vi "CSM - Mermaid - DebugTool.vi"() -> ()   [LabVIEW 2020]
doc: "Show CSM relationship Graph with mermaid"
uses:
  <vilib>/sklein/WebView2 XControl/WebView2 XControl/WebView2 Control.xctl
  <userlib>/_NEVSTOP/Communicable State Machine(CSM)/_Support/Typedef/_CSM_GlobalLog_MSG.ctl
  <userlib>/_NEVSTOP/Communicable State Machine(CSM)/_Support/Typedef/_CSM_Response Source Message.ctl
  <userlib>/_NEVSTOP/Communicable State Machine(CSM)/_Support/Typedef/_CSM_GlobalLog_MSG_TYPE.ctl
  <userlib>/_NEVSTOP/Communicable State Machine(CSM)/_tool/_debugConsole/_BroadcastDef.ctl
  <userlib>/_NEVSTOP/Communicable State Machine(CSM)/AdvanceAPI/CSM - Convert Error to Argument.vi
  <userlib>/_NEVSTOP/Communicable State Machine(CSM)/_Support/GlobalEvent/GEvt-Generate with Rule Check.vi
  <userlib>/_NEVSTOP/Communicable State Machine(CSM)/_Support/GlobalEvent/Cache-GEvt Refs.vi
  <userlib>/_NEVSTOP/Communicable State Machine(CSM)/AdvanceAPI/CSM - Make String Arguments Safe.vi
  <userlib>/_NEVSTOP/Communicable State Machine(CSM)/_Support/ChangeFlag/FlagInstance-GEvt Refs.vi
  <userlib>/_NEVSTOP/Communicable State Machine(CSM)/AdvanceAPI/CSM - Keywords.vi
  <userlib>/_NEVSTOP/Communicable State Machine(CSM)/_Support/ChangeFlag/ChangeFlag-Read.vi
  <userlib>/_NEVSTOP/Communicable State Machine(CSM)/_Polymophic/Add State(s) to Queue By BOOL(Element).vi
  <userlib>/_NEVSTOP/Communicable State Machine(CSM)/_Support/ChangeFlag/ChangeFlagDB.vi
  <userlib>/_NEVSTOP/Communicable State Machine(CSM)/_Support/GlobalEvent/FGV-GlobalEventRef(lvlibp).vi
  <userlib>/_NEVSTOP/Communicable State Machine(CSM)/_Support/GlobalEvent/FGV-GlobalEventQueues(lvlibp).vi
  <userlib>/_NEVSTOP/Communicable State Machine(CSM)/_Support/GlobalEvent/GEvt-Valid Subscribers.vi
  <userlib>/_NEVSTOP/Communicable State Machine(CSM)/_Support/GlobalEvent/LogFilter/LogFilter - Check.vi
  <userlib>/_NEVSTOP/Communicable State Machine(CSM)/_csmHelper/API/Create From VI Reference.vi
  <userlib>/_NEVSTOP/Communicable State Machine(CSM)/_csmHelper/API/Destroy.vi
  <userlib>/_NEVSTOP/Communicable State Machine(CSM)/_Support/GlobalEvent/LogFilter/LogFilter.lvclass
  <userlib>/_NEVSTOP/Communicable State Machine(CSM)/Communicable State Machine.lvlib
  _support/CSM Mermaid Support.lvlib
  <userlib>/_NEVSTOP/Communicable State Machine(CSM)/_csmHelper/CSM-Helper.lvclass
  <userlib>/_NEVSTOP/Communicable State Machine(CSM)/_tool/_file/csm-file-support.lvlib
  <userlib>/_NEVSTOP/Communicable State Machine(CSM)/_tool/_ui/csm-ui-support.lvlib
  <userlib>/_NEVSTOP/Communicable State Machine(CSM)/_tool/_csmlite/_csmlite.lvlib
  <userlib>/_NEVSTOP/Communicable State Machine(CSM)/_tool/_debugConsole/DebugConsole.lvlib
panel:
  in  "CSM":string(combo)
  in  "Search Button":bool
  in  "Draw Mermaid":bool
  in  "Type":T1(ring)
  in  "Tab":T2(tab)
  out "mermaid string":string
  in  "WebView2 Control":string(xcontrol)
  # "https://mermaid.live/"
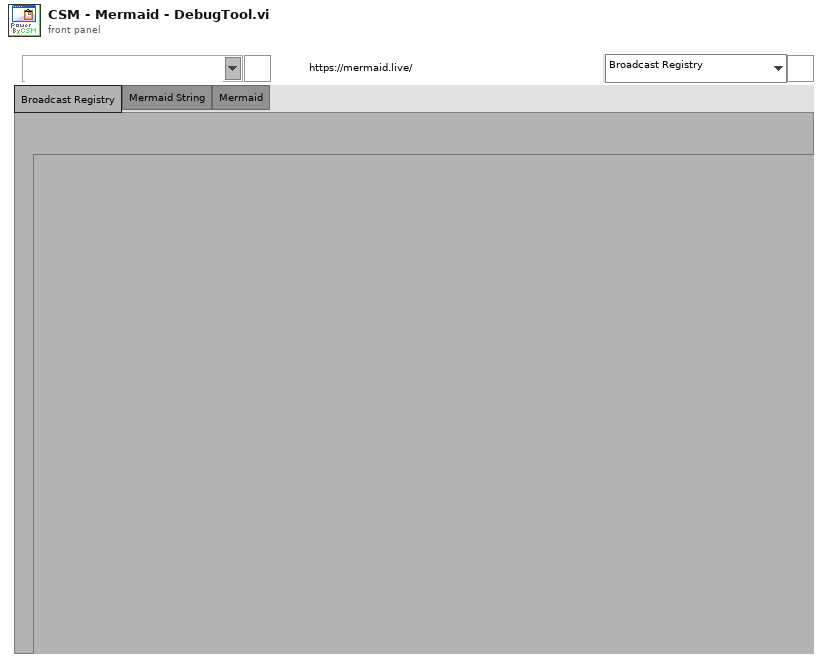
[diagram p1: front panel]
types:
  T1 = enum16{"Broadcast Registry", "CSM Interface", "CSM All Interfaces"}
  T2 = enum32{"Broadcast Registry", "Mermaid String", "Mermaid"}
  T3 = typedef "Communicable State Machine.lvlib/_CSM_GlobalLog_MSG.ctl" = cluster{"Name (\"\" to Use UUID)":string, "Current State":string, "Arguments":string, "Source Message":T4, "Source Module":string, "Complete(T)/Start(F)":bool, "LogType":T5, "Time Stamp":timestamp}
  T4 = typedef "Communicable State Machine.lvlib/_CSM_Response Source Message.ctl" = cluster{"‘State":string, "’Arguments":string, "’Error":errorcluster}
  T5 = typedef "Communicable State Machine.lvlib/_CSM_GlobalLog_MSG_TYPE.ctl" = enum16{"User Log", "State Change", "Status", "Interrupt", "Register", "Unregister", "Error Log", "Module Created", "Module Destroyed", "Async Message", "No-Rep Async Message", "Sync Message"}
  T6 = enum32{"Broadcast Registry", "Mermaid String", "Mermaid", "Error History"}
  T7 = enum32{"Invalid", "Standard", "Closed", "Hidden", "Minimized", "Maximized"}
  T8 = enum32{"invalid app kind", "Development System", "Run Time System", "Student Edition", "Embedded LabVIEW", "Evaluation", "Custom"}
  T9 = typedef "DebugConsole.lvlib/_BroadcastDef.ctl" = enum16{"<no action>", "Macro: Exit", "CSM: Module List Changed", "CSM: Scripts Changed", "CSM: Registration Changed", "CSM: Module Selected", "CSM: Message Excuted", "CSM: Broadcast Excuted", "CSM: Registration Action Excuted", "UI: Try to Change Command"}
  T10 = cluster{"Event Registration Refnum":refnum<event-registration>, "Event Registration Refnum":refnum<event-registration>}
  T11 = cluster{"Shift":bool, "Ctrl":bool, "Alt":bool, "Cmd":bool, "Opt":bool}
  T12 = cluster{"Core":cluster{"Current VI Reference":refnum<vi>, "Close Panel on Exit?":bool}, "Toolbar.Advance":refnum<vi>[], "LoggerWatchDogQueue":refnum<queue>, "LogFile":path, "Mermaid":cluster{"Template":string, "output path":path, "string":string}}
  T13 = cluster{"Template":string, "output path":path, "string":string}
  T14 = cluster{"Current VI Reference":refnum<vi>, "Close Panel on Exit?":bool}
  T15 = cluster{"Left":i32, "Right":i32, "Height":i32, "Width":i32}
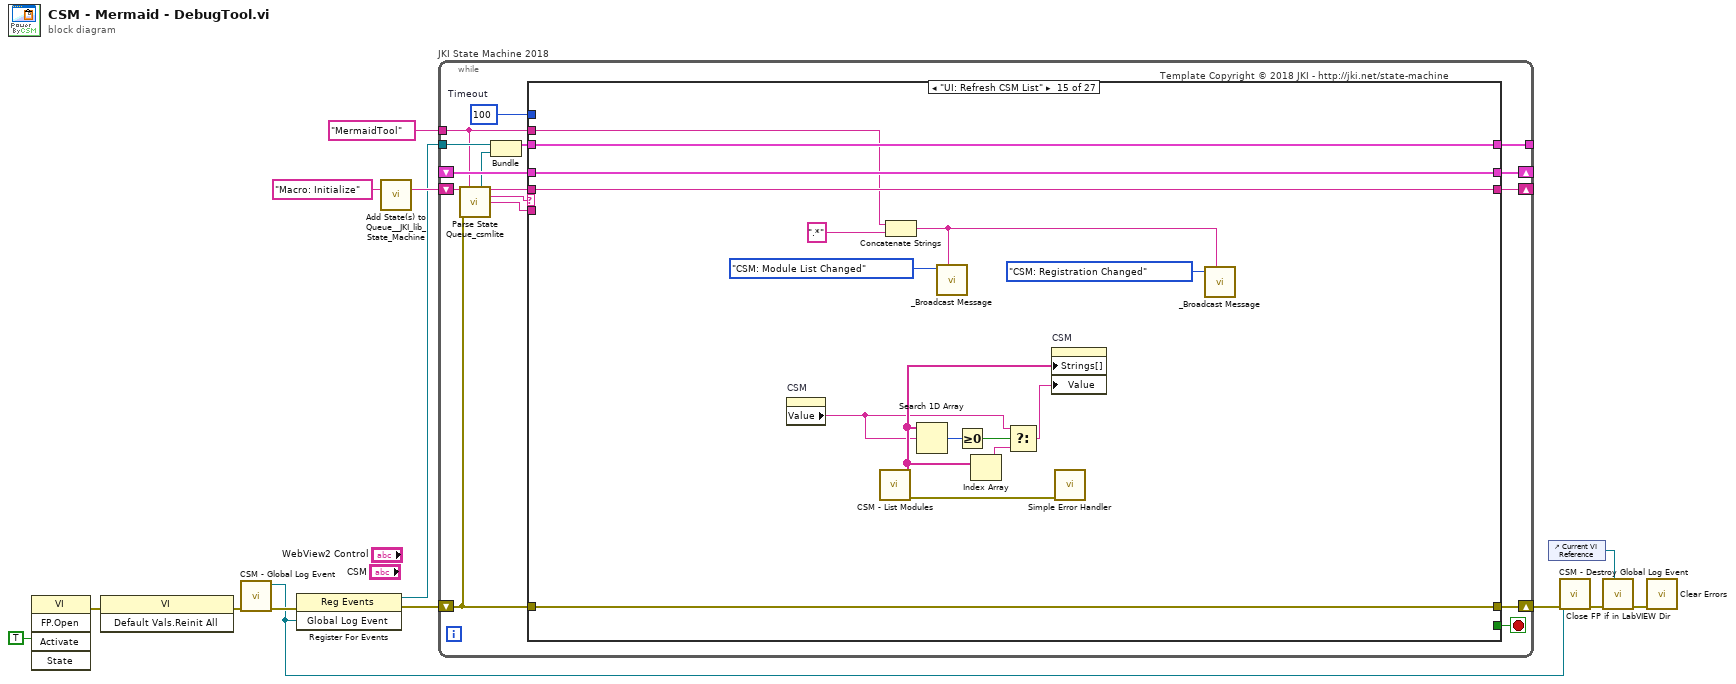
[diagram p0: block diagram]
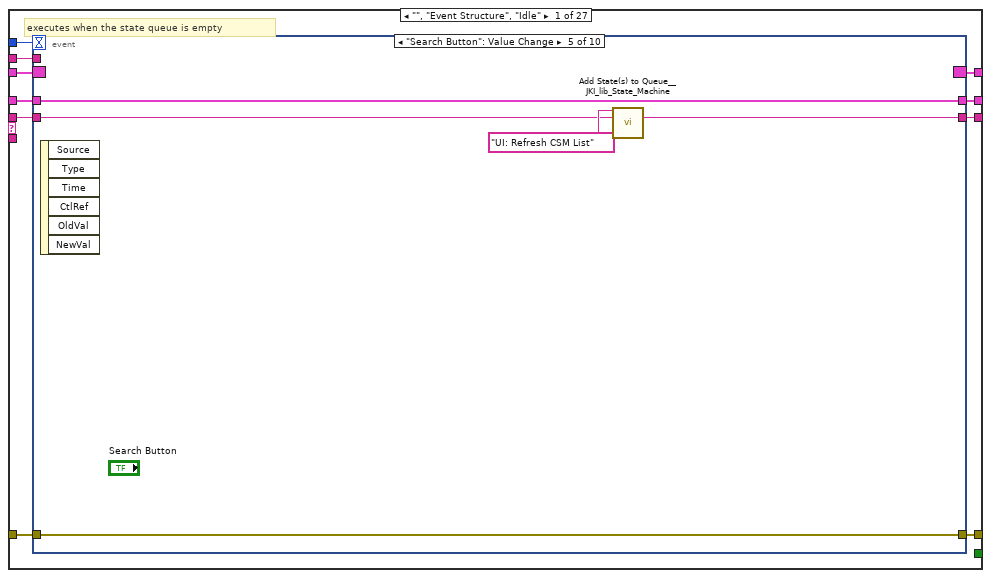
[diagram p2: hidden frame]
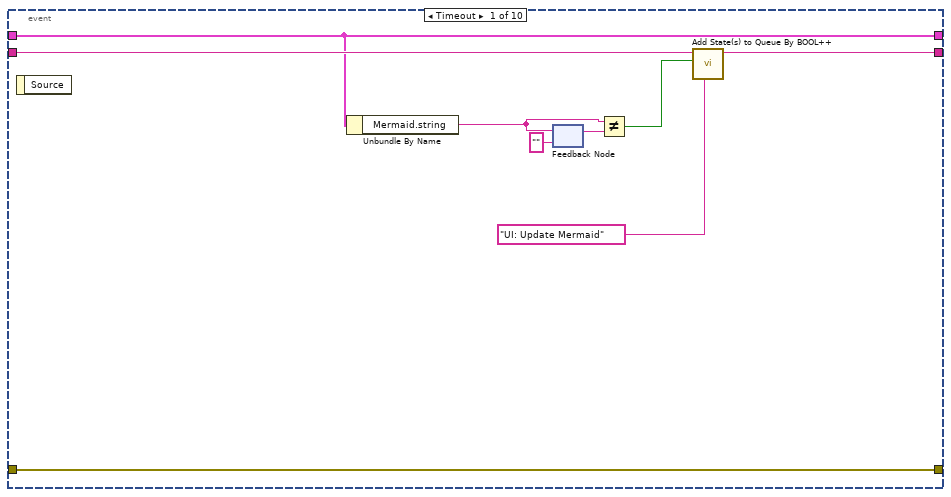
[diagram p3: hidden frame]
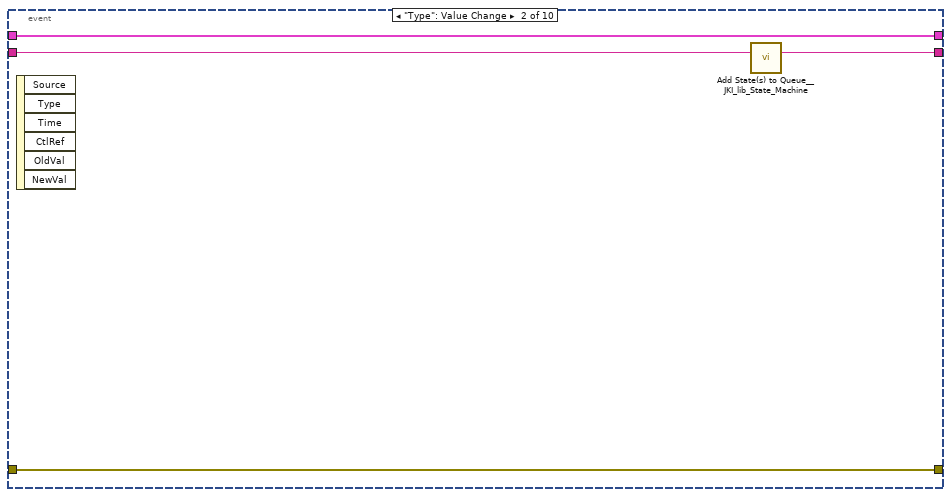
[diagram p4: hidden frame]
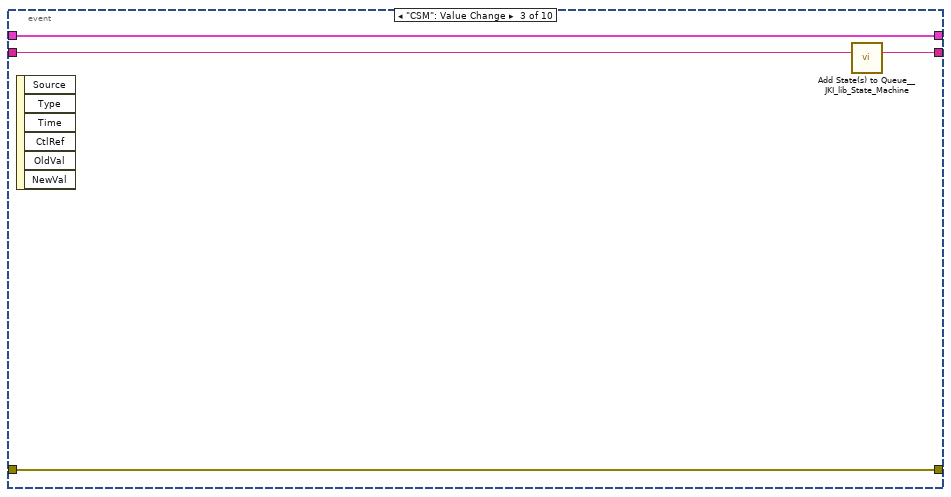
[diagram p5: hidden frame]
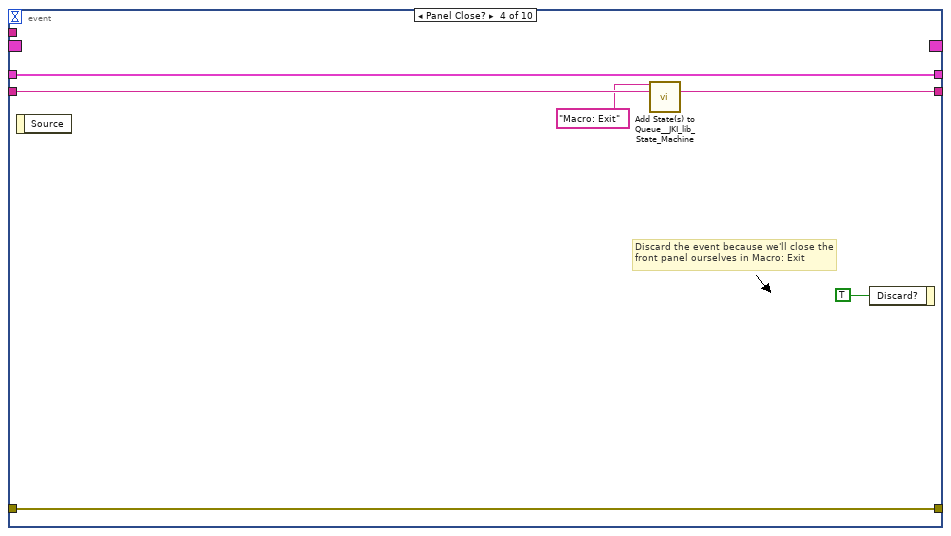
[diagram p6: hidden frame]
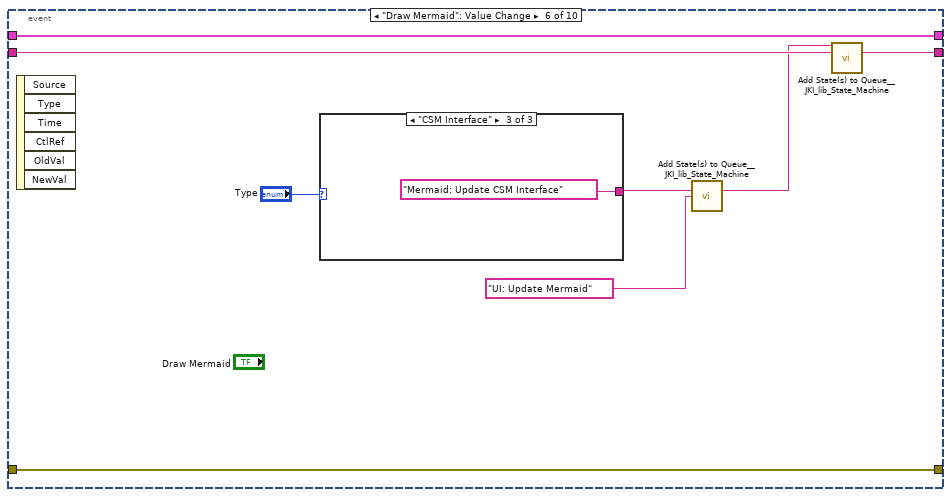
[diagram p7: hidden frame]
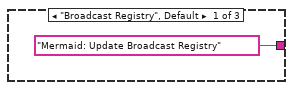
[diagram p8: hidden frame]
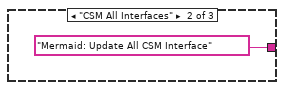
[diagram p9: hidden frame]
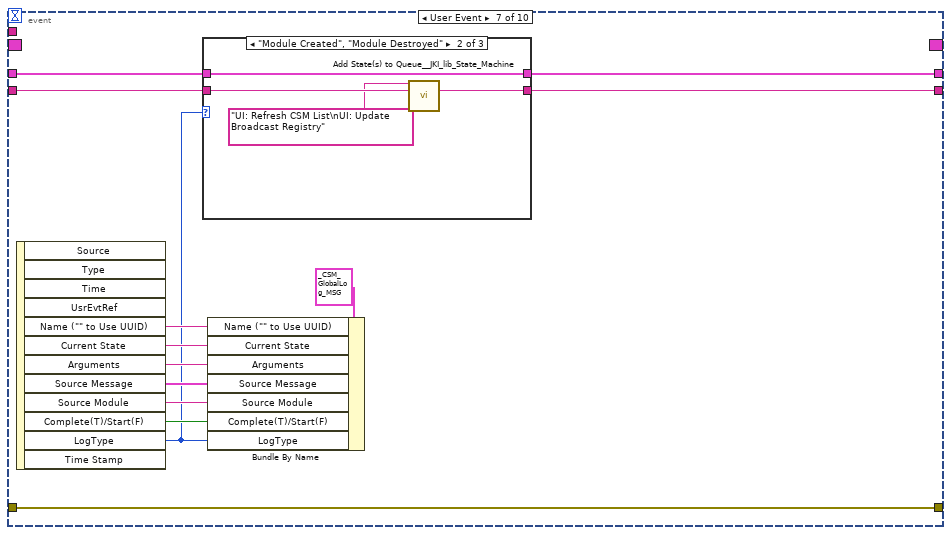
[diagram p10: hidden frame]
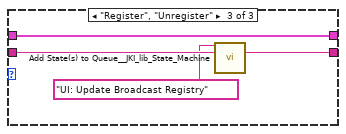
[diagram p12: hidden frame]
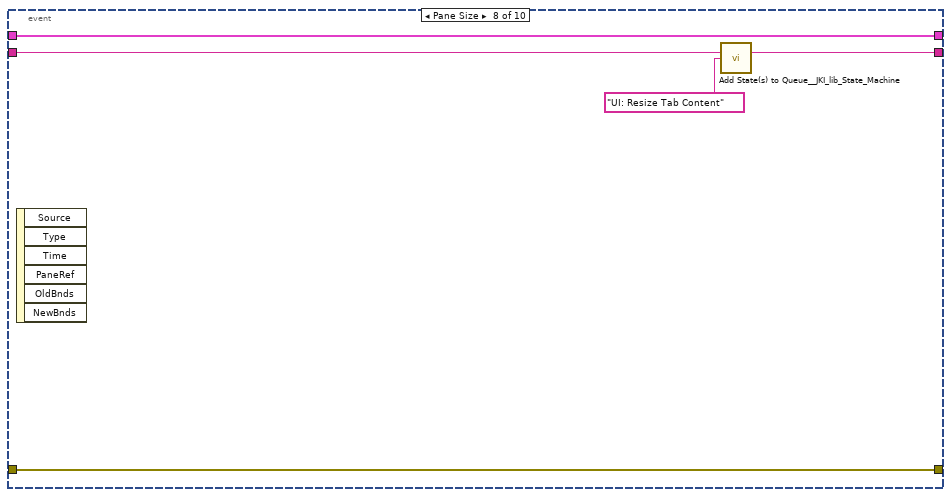
[diagram p13: hidden frame]
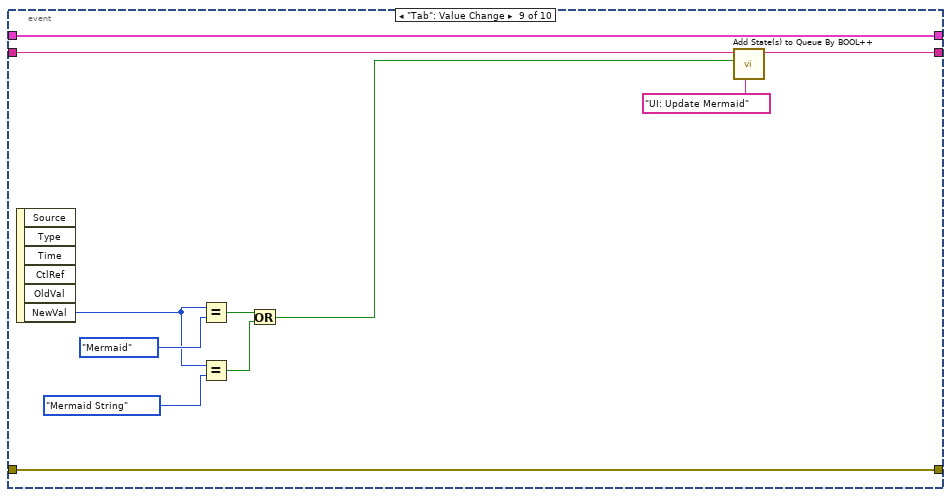
[diagram p14: hidden frame]
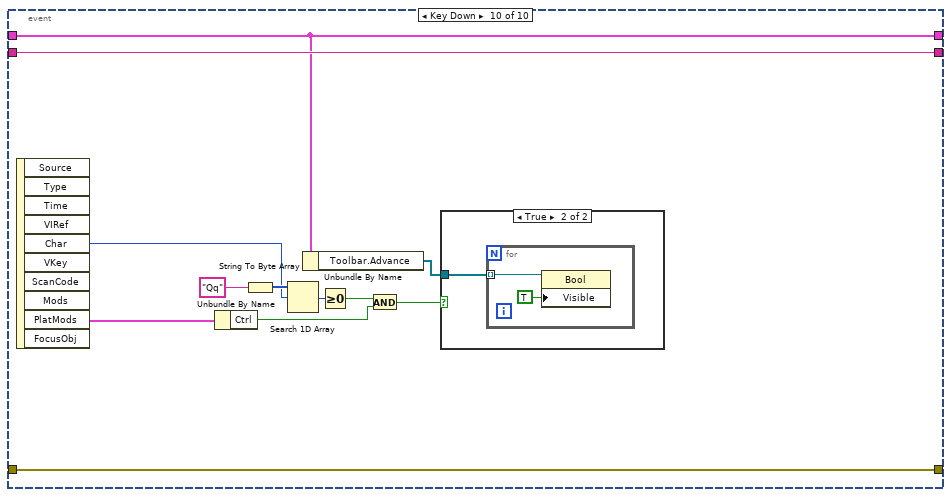
[diagram p15: hidden frame]
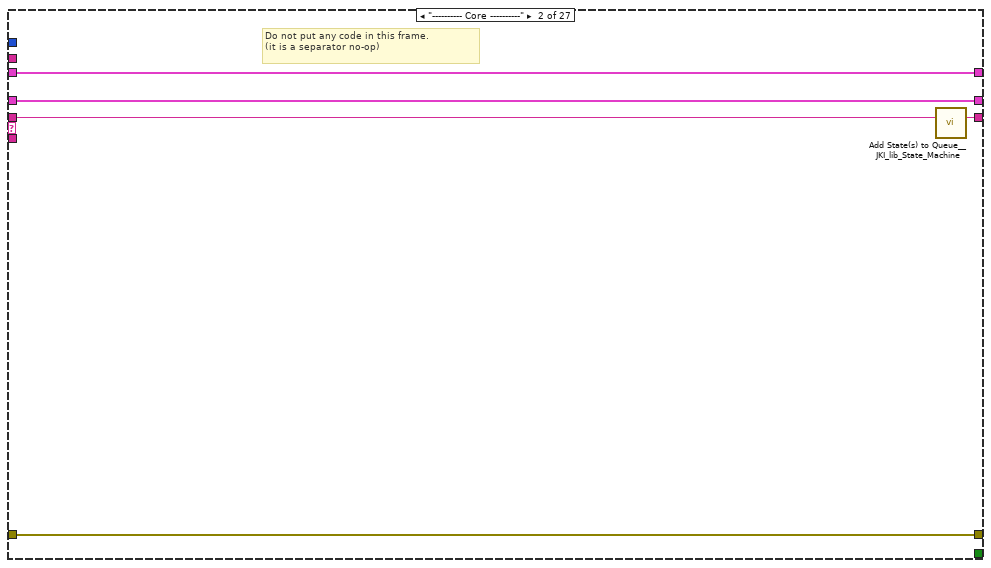
[diagram p17: hidden frame]
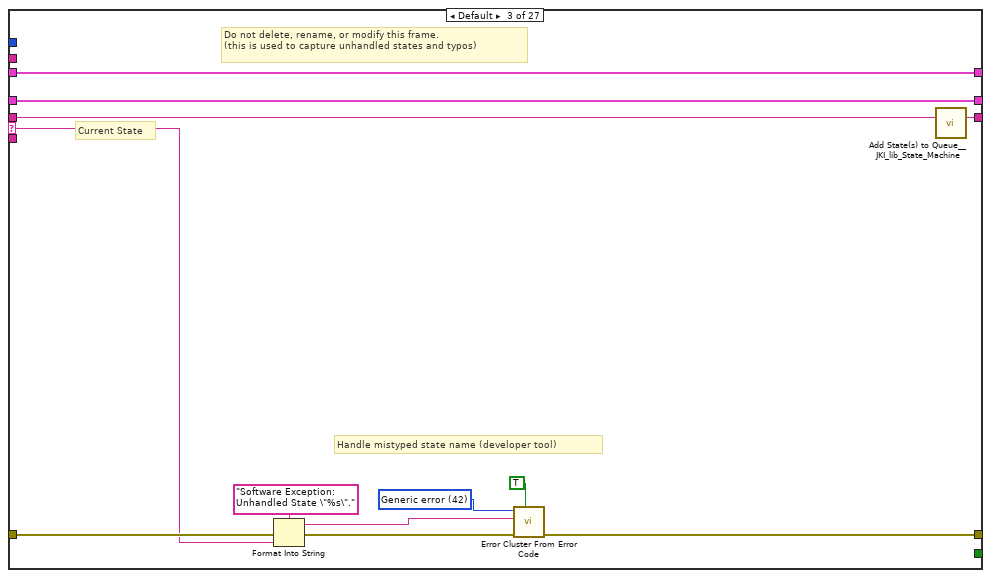
[diagram p18: hidden frame]
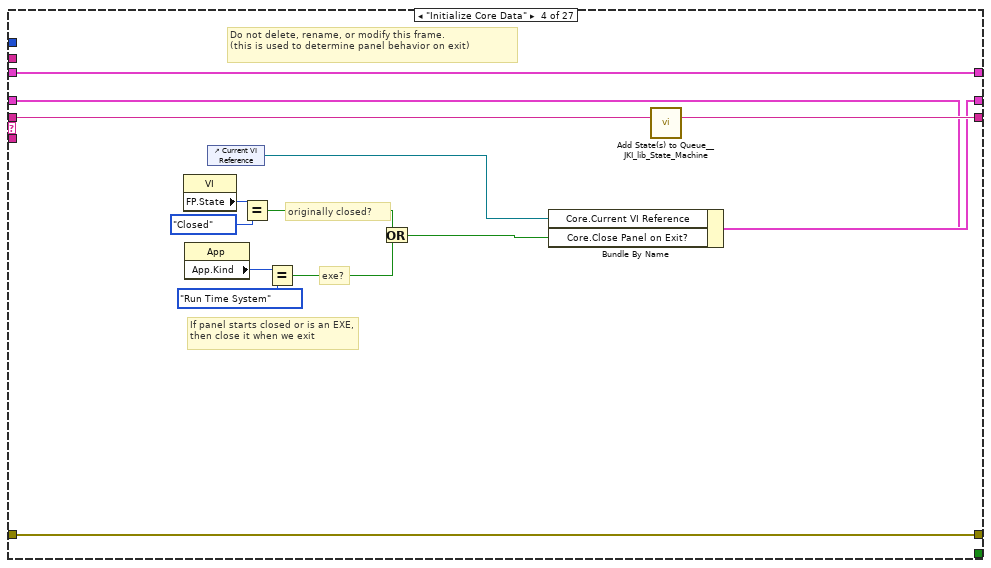
[diagram p19: hidden frame]
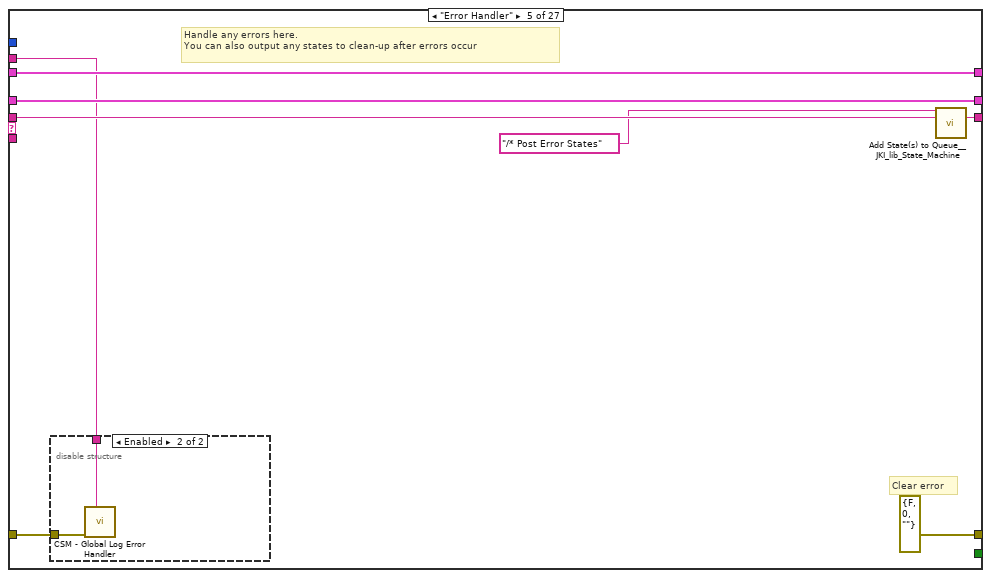
[diagram p20: hidden frame]
diagram:
  n1 = invoke class="VI" method="FP.Open"("Activate"=TRUE ("Activate?")) -> (error out=w13:errorcluster)  [unwired: 4 in, 4 out]
  n2 = invoke class="VI" method="Default Vals.Reinit All"(error in=w13) -> (error out=w8:errorcluster)  [unwired: 2 in, 2 out]
  n3 = call <userlib>:"CSM - Global Log Event.vi"("Error In"=w8) -> ("error out"=w12:errorcluster, "Global Log Event"=w11:refnum<user-event>)  [unwired: 9 in]
  n4 = register-events(error in=w12, w11) -> (reference out=w6:refnum<event-registration>, error out=w7:errorcluster)  [unwired: 1 in]
  n5 = call <vilib>:"Add State(s) to Queue__JKI_lib_State_Machine.vi"("State(s) in (\"\")"="Macro: Initialize") -> ("States Out"=w10:string)  [unwired: 14 in]
  n6 = while "JKI State Machine 2018" {
    shift-right: [w23] -> _
    shift-left: _ -> [w22]
    shift-right: [w26] -> w5
    shift-left: w7 -> [w20]
    shift-right: [w25] -> _
    shift-left: w10 -> [w27]
    tunnel: "MermaidTool" ("Current Module(\"\" to generate a ID)") -> [w17]
    tunnel: w6 -> [w19]
    tunnel: [w18] -> _
    stop <- w24 stop-if-true
    w21 = 100  # Timeout
    # "Template Copyright © 2018 JKI - http://jki.net/state-machine"
    n7 = call <userlib>:"Parse State Queue_csmlite.vi"("State Queue"=w27, "Current Module(\"\" to generate an ID)"=w17, "Error In (no error)"=w20) -> ("Event Registration Refnum"=w15:refnum<event-registration>, "Remaining States"=w29:string, "Current State"=w30:string, "Arguments"=w28:string)  [unwired: 9 in]
    n8 = Bundle("Event Registration Refnum"=w19, "Event Registration Refnum"=w15) -> (w16:T10)  [unwired: 1 in]
    n9 = case shown="\"UI: Refresh CSM List\"" w30 {
      selector: w30 -> [_ _ w140 _ _ _ _ _ _ _ _ _ _ _ _ _ _ _ _ _ _ _ _ _ _ _ _]
      tunnel: w29 -> [w40 w138 w144 w164 w172 w181 w186 w213 w223 w231 w236 w241 w250 w262 w342 w348 w361 w378 w399 w408 w414 w434 w441 w444 w462 w493 w510]
      tunnel: w28 -> [_ _ _ _ _ _ _ _ _ _ _ _ w245 w256 _ _ _ _ _ _ _ _ _ _ _ _ _]
      tunnel: w22 -> [w38 w135 w142 w157 w169 w176 w183 _ w222 w226 w233 w238 w248 w258 w341 w351 w359 w376 w398 w405 w411 w419 w440 w448 w461 w492 w509]
      tunnel: [w37 w136 w146 w161 errorcluster {"status"=FALSE, "code"=0, "source"=""} ("error out") w179 w184 w210 w220 w224 w234 _ w246 w259 w343 w352 w362 w379 w400 w406 w412 w432 w442 w449 w450 w483 w511] -> w26
      tunnel: w20 -> [w36 w136 w145 w161 w168 w179 w184 w210 w220 w228 w234 _ w247 w260 w343 w352 w362 w379 w400 w406 w412 w432 w442 w449 w450 w483 w511]
      tunnel: [w39 w137 w143 w163 w171 w180 w185 w212 w223 w230 w235 w240 w249 w261 w342 w349 w361 w378 w399 w407 w413 w433 w441 w445 w462 w493 w510] -> w25
      tunnel: [_ _ _ _ _ TRUE _ _ _ _ _ _ _ _ _ _ _ _ _ _ _ _ _ _ _ _ _] -> w24
      tunnel: [w35 w135 w142 w162 w169 w176 w183 w197 w222 w226 w233 w238 w248 w258 w341 w351 w359 w376 w398 w405 w411 w419 w440 w446 w459 w490 w509] -> w23
      tunnel: w21 -> [w34 _ _ _ _ _ _ _ _ _ _ _ _ _ _ _ _ _ _ _ _ _ _ _ _ _ _]
      tunnel: w16 -> [w33 w134 w139 w151 w166 w177 w182 w208 w221 w225 w232 w239 w244 w255 w340 w350 w360 w377 w397 w404 w409 w425 w439 w447 w460 w491 w508]
      tunnel: [w32 w134 w139 w151 w166 w177 w182 w208 w221 w225 w232 w239 w244 w255 w340 w350 w360 w377 w397 w404 w409 w425 w439 w447 w460 w491 w508] -> w18
      tunnel: w17 -> [w31 _ _ _ w165 _ _ _ _ _ _ _ _ _ w330 w345 _ _ _ _ _ w415 _ _ w457 w488 w494]
      frame "", "Event Structure", "Idle" {
        # "executes when the state queue is empty"
        n10 = event shown="[4] \"Search Button\": Value Change" {
          selector: w33 -> [_ _ _ _ _ _ _ _ _ _]
          dyn-events: [_ _ _ _ _ _ _ _ _ _] -> w32
          timeout: w34 -> [_ _ _ _ _ _ _ _ _ _]
          tunnel: w40 -> [w49 w50 w54 w63 w65 w72 w84 w104 w115 w130]
          tunnel: [w48 w51 w55 w62 w64 w73 w83 w105 w116 w130] -> w39
          tunnel: w38 -> [w45 w52 w56 w60 w68 w75 w80 w106 w117 w121]
          tunnel: [w47 w53 w57 w61 w67 w76 w92 w107 w118 w129] -> w37
          tunnel: w36 -> [w47 w53 w57 w61 w67 w76 w92 w107 w118 w129]
          tunnel: [w45 w52 w56 w60 w68 w75 w81 w106 w117 w121] -> w35
          tunnel: w31 -> [_ _ _ _ _ _ _ _ _ _]
          event Timeout {
            n11 = event-data() -> ()  [unwired: 1 in, 1 out]
            n12 = Unbundle By Name(w45) -> ("Mermaid.string"=w42:string)
            n13 = feedback #1("" ("string")) -> (w43:string)
            n14 = feedback-in #1(w42) -> ()
            n15 = Not Equal?(x=w42, y=w43) -> (x != y?=w41:bool)
            n16 = call-poly <userlib>:"Add State(s) to Queue By BOOL++.vi"("TRUE (\"\")"="UI: Update Mermaid" ("State(s) in Front (\"\")"), "Condition"=w41, "State Queue (\"\")"=w49) -> ("Remaining States"=w48:string)  [unwired: 8 in]
          }
          event "Type": Value Change {
            n17 = event-data() -> ()  [unwired: 1 in, 6 out]
            n18 = call <vilib>:"Add State(s) to Queue__JKI_lib_State_Machine.vi"("State(s) in (\"\")"=w50) -> ("States Out"=w51:string)  [unwired: 14 in]
          }
          event "CSM": Value Change {
            n19 = event-data() -> ()  [unwired: 1 in, 6 out]
            n20 = call <vilib>:"Add State(s) to Queue__JKI_lib_State_Machine.vi"("State(s) in (\"\")"=w54) -> ("States Out"=w55:string)  [unwired: 14 in]
          }
          event Panel Close? {
            # "Discard the event because we'll close the front panel ourselves in Macro: Exit"
            n21 = event-data() -> ()  [unwired: 1 in, 1 out]
            n22 = call <vilib>:"Add State(s) to Queue__JKI_lib_State_Machine.vi"("State(s) in Front (\"\")"="Macro: Exit", "State(s) in (\"\")"=w63) -> ("States Out"=w62:string)  [unwired: 13 in]
            n23 = event-data("Discard?"=TRUE) -> ()  [unwired: 1 in, 1 out]
          }
          event "Search Button": Value Change {
            n24 = event-data() -> ()  [unwired: 1 in, 6 out]
            n25 = call <vilib>:"Add State(s) to Queue__JKI_lib_State_Machine.vi"("State(s) in Front (\"\")"="UI: Refresh CSM List" ("State(s) in Front (\"\")"), "State(s) in (\"\")"=w65) -> ("States Out"=w64:string)  [unwired: 13 in]
          }
          event "Draw Mermaid": Value Change {
            n26 = event-data() -> ()  [unwired: 1 in, 6 out]
            n27 = case shown="\"CSM Interface\"" "Type" {
              tunnel: ["Mermaid: Update Broadcast Registry" ("State(s) in Front (\"\")") "Mermaid: Update All CSM Interface" ("State(s) in Front (\"\")") "Mermaid: Update CSM Interface" ("State(s) in Front (\"\")")] -> w71
              frame "Broadcast Registry", Default {
              }
              frame "CSM All Interfaces" {
              }
              frame "CSM Interface" {
              }
            }
            n28 = call <vilib>:"Add State(s) to Queue__JKI_lib_State_Machine.vi"("State(s) in (\"\")"=w71, "State(s) at Back (\"\")"="UI: Update Mermaid" ("State(s) in Front (\"\")")) -> ("States Out"=w69:string)  [unwired: 13 in]
            n29 = call <vilib>:"Add State(s) to Queue__JKI_lib_State_Machine.vi"("State(s) in Front (\"\")"=w69, "State(s) in (\"\")"=w72) -> ("States Out"=w73:string)  [unwired: 13 in]
          }
          event User Event {
            n30 = event-data() -> ("Name (\"\" to Use UUID)"=w90:string, "Current State"=w89:string, "Arguments"=w88:string, "Source Message"=w87:T4, "Source Module"=w86:string, "Complete(T)/Start(F)"=w85:bool, "LogType"=w82:T5)  [unwired: 1 in, 5 out]
            n31 = case shown="\"Module Created\", \"Module Destroyed\"" w82 {
              tunnel: w84 -> [w94 w98 w102]
              tunnel: [w94 w97 w101] -> w83
              tunnel: [w93 w95 w99] -> w81
              tunnel: w80 -> [w93 w95 w99]
              frame "User Log", Default {
              }
              frame "Module Created", "Module Destroyed" {
                n32 = call <vilib>:"Add State(s) to Queue__JKI_lib_State_Machine.vi"("State(s) in Front (\"\")"="UI: Refresh CSM List\nUI: Update Broadcast Registry" ("State(s) in Front (\"\")"), "State(s) in (\"\")"=w98) -> ("States Out"=w97:string)  [unwired: 13 in]
              }
              frame "Register", "Unregister" {
                n33 = call <vilib>:"Add State(s) to Queue__JKI_lib_State_Machine.vi"("State(s) in Front (\"\")"="UI: Update Broadcast Registry" ("State(s) in Front (\"\")"), "State(s) in (\"\")"=w102) -> ("States Out"=w101:string)  [unwired: 13 in]
              }
            }
            n34 = Bundle By Name(cluster=T3 {"Name (\"\" to Use UUID)"="", "Current State"="", "Arguments"="", "Source Message"={"‘State"="", "’Arguments"="", "’Error"={"status"=FALSE, "code"=0, "source"=""}}, "Source Module"="", "Complete(T)/Start(F)"=FALSE, "LogType"=enum."State Change", "Time Stamp"=timestamp(0 s since 1904-01-01)} ("Cross CSM Data"), "Name (\"\" to Use UUID)"=w90, "Current State"=w89, "Arguments"=w88, "Source Message"=w87, "Source Module"=w86, "Complete(T)/Start(F)"=w85, "LogType"=w82) -> ()  [unwired: 1 out]
          }
          event Pane Size {
            n35 = event-data() -> ()  [unwired: 1 in, 6 out]
            n36 = call <vilib>:"Add State(s) to Queue__JKI_lib_State_Machine.vi"("State(s) in (\"\")"=w104, "State(s) at Back (\"\")"="UI: Resize Tab Content" ("State(s) in Front (\"\")")) -> ("States Out"=w105:string)  [unwired: 13 in]
          }
          event "Tab": Value Change {
            n37 = event-data() -> ("NewVal"=w109:T2)  [unwired: 1 in, 5 out]
            n38 = Equal?(x=w109, y=T6."Mermaid") -> (x = y?=w112:bool)
            n39 = Equal?(x=w109, y=T6."Mermaid String") -> (x = y?=w108:bool)
            n40 = Or(x=w112, y=w108) -> (x .or. y?=w111:bool)
            n41 = call-poly <userlib>:"Add State(s) to Queue By BOOL++.vi"("TRUE (\"\")"="UI: Update Mermaid" ("TRUE(\"\")"), "Condition"=w111, "State Queue (\"\")"=w115) -> ("Remaining States"=w116:string)  [unwired: 8 in]
          }
          event Key Down {
            n42 = event-data() -> ("Char"=w119:i16, "PlatMods"=w124:T11)  [unwired: 1 in, 8 out]
            n43 = Unbundle By Name(w124) -> ("Ctrl"=w123:bool)
            n44 = String To Byte Array(string="Qq") -> (unsigned byte array=w126:u8[])
            n45 = Search 1D Array(1D array=w126, element=w119) -> (index of element=w127:i32)  [unwired: 1 in]
            n46 = Unbundle By Name(w121) -> ("Toolbar.Advance"=w120:refnum<vi>[])
            n47 = Greater Or Equal To 0?(x=w127) -> (x >= 0?=w128:bool)
            n48 = And(x=w128, y=w123) -> (x .and. y?=w122:bool)
            n49 = case shown="True" w122 {
              tunnel: w120 -> [_ w131]
              frame False {
              }
              frame True {
                n50 = for {
                  tunnel: w131 -> [w133] mode=indexing
                  n51 = property class="Bool"(reference=w133, "Visible"=TRUE) -> ()  [unwired: 1 in, 2 out]
                }
              }
            }
          }
        }
      }
      frame "---------- Core ----------" {
        # "Do not put any code in this frame.\n(it is a separator no-op)"
        n52 = call <vilib>:"Add State(s) to Queue__JKI_lib_State_Machine.vi"("State(s) in (\"\")"=w138) -> ("States Out"=w137:string)  [unwired: 14 in]
      }
      frame Default {
        w149 = 42 items=["No error", "Argument error", "Memory is full", "Out of zone", "End of file", "File already open", "Generic file I/O error", "File not found", "File permission error", "Disk is full", "Duplicate path", "Too many files open", "System feature not enabled", "Resource file not found", "Cannot add resource", "Resource not found", "Image not found", "Image memory error", "Pen does not exist", "Config type invalid", "Config token not found", "Config parse error", "Config memory error", "Bad external code format", "Bad external code offset", "External code not present", "Null window", "Destroy window error", "Null menu", "Print aborted", "Bad print record", "Print driver error", "Windows error during printing", "Memory error during printing", "Print dialog error", "Generic print error", "Invalid device refnum", "Device not found", "Device parameter error", "Device unit error", "Cannot open device", "Device call aborted", "Generic error", "Cancelled by user", "Object ID too low", "Object ID too high", "Object not in heap", "Unknown heap", "Unknown object (invalid DefProc)", "Unknown object (DefProc not in table)", "Message out of range", "Invalid (null) method", "Unknown message", "Manager call not supported", "Bad address", "Network operation in progress", "Network operation timed out", "Connection is busy", "Network attribute not supported", "Network error", "Address in use", "System out of memory", "Connection aborted", "Connection refused", "Not connected", "Already connected", "Connection closed", "Initialization error (interapplication manager)", "Bad occurrence", "Wait on unbound occurrence handler", "Occurrence queue overflow", "Datalog type conflict", "Unused", "Unrecognized type (interapplication manager)", "Memory corrupt", "Failed to make temporary DLL", "Old CIN version", "Drag socket not found", "Failed to load drop-object", "Failed to register OLE object", "Failed to release OLE object", "Format specifier type mismatch", "Unknown format specifier", "Too few format specifiers", "Too many format specifiers", "Scan failed", "Newer CIN version", "Error converting to variant", "Runtime menu error", "Password tampered", "Variant attribute not found", "Incompatible variant data type", "Event data is not available", "Event Store is not present", "Occurrence is not found", "Event Queue is not created", "Event info is not available", "Refnum passed is NULL", "Error retrieving Class GUID", "Error retrieving CoClass GUID", "Error retrieving TypeLib GUID.", "Bad built application magic bytes.", "Specific driver is different from the specific driver associated with the Logical Name.", "There is no session opened to the class driver.", "Max Error", "MAX - Error with config objects", "MAX - Error loading configuration", "MAX - Group not supported"]
        # "Current State"
        # "Do not delete, rename, or modify this frame.\n(this is used to capture unhandled states and typos)"
        # "Handle mistyped state name (developer tool)"
        n53 = Format Into String(format string="Software Exception: Unhandled State \"%s\"." ("message"), error in=w145, w140) -> (resulting string=w148:string, error out=w147:errorcluster)  [unwired: 1 in]
        n54 = call <vilib>:"Error Cluster From Error Code.vi"("show call chain? (False)"=TRUE, "error in (no error)"=w147, "error message (\"\")"=w148, "error code (0)"=w149) -> ("error out"=w146:errorcluster)  [unwired: 5 in]
        n55 = call <vilib>:"Add State(s) to Queue__JKI_lib_State_Machine.vi"("State(s) in (\"\")"=w144) -> ("States Out"=w143:string)  [unwired: 14 in]
      }
      frame "Initialize Core Data" {
        # "Do not delete, rename, or modify this frame.\n(this is used to determine panel behavior on exit)"
        # "originally closed?"
        # "exe?"
        # "If panel starts closed or is an EXE, then close it when we exit"
        n56 = property class="VI"() -> ("FP.State"=w154:T7)  [unwired: 2 in, 2 out]
        n57 = property class="App"() -> ("App.Kind"=w160:T8)  [unwired: 2 in, 2 out]
        n58 = control-ref of="Current VI Reference"() -> (w155:refnum<vi>)
        n59 = Equal?(x=w154, y=T7."Closed" ("Front Panel Window:State")) -> (x = y?=w152:bool)
        n60 = Equal?(x=w160, y=T8."Run Time System" ("Application:Kind")) -> (x = y?=w158:bool)
        n61 = Or(x=w152, y=w158) -> (x .or. y?=w156:bool)
        n62 = Bundle By Name(cluster=w157, "Core.Current VI Reference"=w155, "Core.Close Panel on Exit?"=w156) -> (w162:T12)
        n63 = call <vilib>:"Add State(s) to Queue__JKI_lib_State_Machine.vi"("State(s) in (\"\")"=w164) -> ("States Out"=w163:string)  [unwired: 14 in]
      }
      frame "Error Handler" {
        # "Handle any errors here.\nYou can also output any states to clean-up after errors occur"
        # "Clear error"
        n64 = disable-structure "Diagram Disable Structure" shown="Enabled" {
          disable-tunnel: w168 -> [w173 w175]
          disable-tunnel: w165 -> [_ w174]
          frame Disabled {
            # "Unhandled Error -- Display it"
            n65 = call <vilib>:"General Error Handler.vi"("error in (no error)"=w173) -> ()  [unwired: 10 in, 5 out]
          }
          frame Enabled {
            n66 = call <userlib>:"CSM - Global Log Error Handler.vi"("Place (\"\" to Use VI's Name)"=w174, "Error In"=w175) -> ()  [unwired: 9 in, 1 out]
          }
        }
        n67 = call <vilib>:"Add State(s) to Queue__JKI_lib_State_Machine.vi"("State(s) in Front (\"\")"="/* Post Error States", "State(s) in (\"\")"=w172) -> ("States Out"=w171:string)  [unwired: 13 in]
      }
      frame "Exit" {
        # "Do not put any code in this frame.\n(No errors that occur here will be handled.)"
        n68 = call <vilib>:"Add State(s) to Queue__JKI_lib_State_Machine.vi"("State(s) in (\"\")"=w181) -> ("States Out"=w180:string)  [unwired: 14 in]
      }
      frame "---------- Data ----------" {
        # "Do not put any code in this frame.\n(It is a separator no-op. You can make a copy of this frame to create a new Data frame)"
        n69 = call <vilib>:"Add State(s) to Queue__JKI_lib_State_Machine.vi"("State(s) in (\"\")"=w186) -> ("States Out"=w185:string)  [unwired: 14 in]
      }
      frame "Data: Initialize" {
        w198 = T13 {"Template"="", "output path"=path "", "string"=""}  # Mermaid
        w205 = path ""  # LogFile
        w206 = refnum<queue> refnum  # LoggerWatchDogQueue
        w207 = refnum<vi>[] []  # Toolbar.Advance
        w209 = T14 {"Current VI Reference"=refnum, "Close Panel on Exit?"=FALSE}  # Core
        # "Initialize the shift-register data, here.\n(data names are defined by what you wire into the bundle function)"
        n70 = control-ref of="Current VI Reference"() -> (w195:refnum<vi>)
        n71 = property class="VI"(reference=w195) -> (reference out=w193:refnum<vi>, "VI Path"=w194:path)  [unwired: 1 in, 1 out]
        n72 = Close Reference(reference=w193) -> ()  [unwired: 1 in, 1 out]
        n73 = while {
          shift-right: [w214] -> w192
          shift-left: w194 -> [w216]
          stop <- w218 stop-if-true
          # "is Dir?"
          n74 = Strip Path(path=w216) -> (stripped path=w214:path)  [unwired: 1 out]
          n75 = File/Directory Info(path=w214) -> (directory=w219:bool)  [unwired: 1 in, 6 out]
          n76 = Not A Number/Path/Refnum?(number/path/refnum=w216) -> (NaN/Path/Refnum?=w217:bool)
          n77 = Empty String/Path?(string/path=w216) -> (empty?=w215:bool)
          n78 = Compound Arithmetic op=OR(w219, w217, w215) -> (w218:bool)
        }
        n79 = Build Path(base path=w192, name or relative path=path "" ("Relative path (.)")) -> (appended path=w190:path)
        n80 = call <vilib>:"Recursive File List.vi"("pattern"="Broadcast Registry Mermaid.html" ("pattern(ini by default)"), "Continue Recursing on Error? (F)"=TRUE ("Recrusively(F)"), "Folder Path"=w190) -> ("All Files in Dir"=w189:path[])  [unwired: 4 in, 4 out]
        n81 = Index Array(array=w189) -> (element=w188:path)  [unwired: 1 in]
        n82 = call <userlib>:"uuid.vi"() -> ("UUID"=w199:string)  [unwired: 11 in]
        n83 = Strip Path(path=w188) -> (stripped path=w200:path)  [unwired: 1 out]
        n84 = call <userlib>:"TxtFile Load_CSM.vi"("Path"=w188) -> ("Text"=w187:string)  [unwired: 9 in, 1 out]
        n85 = Concatenate Strings(w199, ".html" ("string")) -> (w201:string)
        n86 = Build Path(base path=w200, name or relative path=w201) -> (appended path=w196:path)
        n87 = Bundle("Core"=w209, "Toolbar.Advance"=w207, "LoggerWatchDogQueue"=w206, "LogFile"=w205, "Mermaid"=w198) -> (w211:T12)  [unwired: 1 in]
        n88 = Bundle By Name(cluster=w211, "Mermaid.Template"=w187, "Mermaid.output path"=w196) -> (w197:T12)
        n89 = call <vilib>:"Add State(s) to Queue__JKI_lib_State_Machine.vi"("State(s) in (\"\")"=w213) -> ("States Out"=w212:string)  [unwired: 14 in]
      }
      frame "Data: Initialize References" {
      }
      frame "Data: Cleanup" {
        # "Cleanup any data and references, here.\n(this is called automatically, by the Macro: Exit)"
        n90 = Unbundle By Name(w226) -> ("Core.Current VI Reference"=w229:refnum<vi>)
        n91 = Close Reference(reference=w229, error in (no error)=w228) -> (error out=w227:errorcluster)
        n92 = Merge Errors(w227) -> (w224:errorcluster)
        n93 = call <vilib>:"Add State(s) to Queue__JKI_lib_State_Machine.vi"("State(s) in (\"\")"=w231) -> ("States Out"=w230:string)  [unwired: 14 in]
      }
      frame "---------- UI ----------" {
        # "Do not put any code in this frame.\n(It is a separator no-op. You can make a copy of this frame to create a new UI frame)"
        n94 = call <vilib>:"Add State(s) to Queue__JKI_lib_State_Machine.vi"("State(s) in (\"\")"=w236) -> ("States Out"=w235:string)  [unwired: 14 in]
      }
      frame "UI: Initialize" {
        # "Initialize the User Interface, here.\n(this is called automatically, by the Macro: Init)"
        n95 = Unbundle By Name(w238) -> ("Toolbar.Advance"=w237:refnum<vi>[])
        n96 = for {
          tunnel: w237 -> [w243] mode=indexing
          n97 = property class="Bool"(reference=w243, "Visible"=FALSE) -> ()  [unwired: 1 in, 2 out]
        }
        n98 = call <vilib>:"Add State(s) to Queue__JKI_lib_State_Machine.vi"("State(s) in (\"\")"=w241) -> ("States Out"=w240:string)  [unwired: 14 in]
      }
      frame "UI: Cursor Set" {
        # "Argument"
        # "Set and Unset Cursor Busy.\n(Usage: \"UI: Cursor Set >> Busy|Idle\")"
        n99 = case shown="\"Idle\", Default" w245 {
          tunnel: w247 -> [w252 w254]
          tunnel: [w251 w253] -> w246
          frame "Idle", Default {
            n100 = call <vilib>:"Unset Busy.vi"("error in (no error)"=w252) -> ("error out"=w251:errorcluster)  [unwired: 10 in]
          }
          frame "Busy" {
            n101 = call <vilib>:"Set Busy.vi"("error in (no error)"=w254) -> ("error out"=w253:errorcluster)  [unwired: 9 in, 1 out]
          }
        }
        n102 = call <vilib>:"Add State(s) to Queue__JKI_lib_State_Machine.vi"("State(s) in (\"\")"=w250) -> ("States Out"=w249:string)  [unwired: 14 in]
      }
      frame "UI: Front Panel State" {
        # "Argument"
        # "Set Front Panel Open or Closed\n(Usage: \"UI: Front Panel State >> Open|Close\")"
        n103 = Unbundle By Name(w258) -> ("Core.Current VI Reference"=w257:refnum<vi>)
        n104 = case shown="\"Minimize\", \"Minimized\"" w256 {
          tunnel: w260 -> [w268 w283 w294 w307 w320]
          tunnel: [w270 w284 w296 w309 w322] -> w259
          tunnel: w257 -> [w269 w281 w295 w308 w321]
          frame "Open", "Standard", Default {
            w263 = T7."Standard" ("State")
            n105 = property class="VI"(reference=w269, error in=w268) -> (reference out=w266:refnum<vi>, error out=w267:errorcluster, "FP.State"=w265:T7)
            n106 = Not Equal?(x=w265, y=w263) -> (x != y?=w264:bool)
            n107 = case shown="True" w264 {
              tunnel: [w274 w276] -> w270
              tunnel: w267 -> [w273 w276]
              tunnel: w266 -> [w272 _]
              tunnel: w263 -> [w271 _]
              frame True {
                n108 = invoke class="VI" method="FP.Open"(reference=w272, error in=w273, "Activate"=TRUE, "State"=w271) -> (error out=w274:errorcluster)  [unwired: 1 in, 4 out]
              }
              frame False {
              }
            }
          }
          frame "Close", "Closed" {
            n109 = property class="VI"(reference=w281, error in=w283) -> (reference out=w280:refnum<vi>, error out=w282:errorcluster, "FP.State"=w278:T7)
            n110 = Not Equal?(x=w278, y=T7."Closed" ("Front Panel Window:State")) -> (x != y?=w277:bool)
            n111 = case shown="True" w277 {
              tunnel: [w285 w288] -> w284
              tunnel: w282 -> [w285 w287]
              tunnel: w280 -> [_ w286]
              frame False {
              }
              frame True {
                n112 = invoke class="VI" method="FP.Close"(reference=w286, error in=w287) -> (error out=w288:errorcluster)  [unwired: 1 in, 2 out]
              }
            }
          }
          frame "Hidden", "Hide" {
            w289 = T7."Hidden" ("State")
            n113 = property class="VI"(reference=w295, error in=w294) -> (reference out=w292:refnum<vi>, error out=w293:errorcluster, "FP.State"=w291:T7)
            n114 = Not Equal?(x=w291, y=w289) -> (x != y?=w290:bool)
            n115 = case shown="True" w290 {
              tunnel: [w300 w301] -> w296
              tunnel: w293 -> [w299 w301]
              tunnel: w292 -> [w298 _]
              tunnel: w289 -> [w297 _]
              frame True {
                n116 = invoke class="VI" method="FP.Open"(reference=w298, error in=w299, "State"=w297) -> (error out=w300:errorcluster)  [unwired: 2 in, 4 out]
              }
              frame False {
              }
            }
          }
          frame "Minimize", "Minimized" {
            w302 = T7."Minimized" ("State")
            n117 = property class="VI"(reference=w308, error in=w307) -> (reference out=w305:refnum<vi>, error out=w306:errorcluster, "FP.State"=w304:T7)
            n118 = Not Equal?(x=w304, y=w302) -> (x != y?=w303:bool)
            n119 = case shown="True" w303 {
              tunnel: [w313 w314] -> w309
              tunnel: w306 -> [w312 w314]
              tunnel: w305 -> [w311 _]
              tunnel: w302 -> [w310 _]
              frame True {
                n120 = invoke class="VI" method="FP.Open"(reference=w311, error in=w312, "State"=w310) -> (error out=w313:errorcluster)  [unwired: 2 in, 4 out]
              }
              frame False {
              }
            }
          }
          frame "Maximize", "Maximized" {
            w315 = T7."Maximized" ("State")
            n121 = property class="VI"(reference=w321, error in=w320) -> (reference out=w318:refnum<vi>, error out=w319:errorcluster, "FP.State"=w317:T7)
            n122 = Not Equal?(x=w317, y=w315) -> (x != y?=w316:bool)
            n123 = case shown="True" w316 {
              tunnel: [w326 w327] -> w322
              tunnel: w319 -> [w325 w327]
              tunnel: w318 -> [w324 _]
              tunnel: w315 -> [w323 _]
              frame True {
                n124 = invoke class="VI" method="FP.Open"(reference=w324, error in=w325, "State"=w323) -> (error out=w326:errorcluster)  [unwired: 2 in, 4 out]
              }
              frame False {
              }
            }
          }
        }
        n125 = call <vilib>:"Add State(s) to Queue__JKI_lib_State_Machine.vi"("State(s) in (\"\")"=w262) -> ("States Out"=w261:string)  [unwired: 14 in]
      }
      frame "UI: Refresh CSM List" {
        n126 = property on="CSM" class="CmbBox"() -> ("Value"=w336:string)  [unwired: 2 in, 2 out]
        n127 = call <userlib>:"CSM - List Modules.vi"() -> ("error out"=w333:errorcluster, "Module Names"=w338:string[])  [unwired: 10 in]
        n128 = Concatenate Strings(w330, ".*") -> (w328:string)
        n129 = Search 1D Array(1D array=w338, element=w336) -> (index of element=w334:i32)  [unwired: 1 in]
        n130 = call <userlib>:"_Broadcast Message.vi"("Module Pattern (support *)"=w328, "Broadcast"=_BroadcastDef."CSM: Module List Changed") -> ()  [unwired: 9 in, 1 out]
        n131 = Greater Or Equal To 0?(x=w334) -> (x >= 0?=w335:bool)
        n132 = Index Array(array=w338) -> (element=w337:string)  [unwired: 1 in]
        n133 = Select(t=w336, s=w335, f=w337) -> (s? t:f=w339:string)
        n134 = property on="CSM" class="CmbBox"("Strings[]"=w338, "Value"=w339) -> ()  [unwired: 2 in, 2 out]
        n135 = call <vilib>:"Simple Error Handler.vi"("error in (no error)"=w333) -> ()  [unwired: 4 in, 5 out]
        n136 = call <userlib>:"_Broadcast Message.vi"("Module Pattern (support *)"=w328, "Broadcast"=_BroadcastDef."CSM: Registration Changed") -> ()  [unwired: 9 in, 1 out]
      }
      frame "UI: Update Broadcast Registry" {
        n137 = Concatenate Strings(w345, ".*") -> (w344:string)
        n138 = call <userlib>:"_Broadcast Message.vi"("Module Pattern (support *)"=w344, "Broadcast"=_BroadcastDef."CSM: Registration Changed") -> ()  [unwired: 9 in, 1 out]
        n139 = call <vilib>:"Add State(s) to Queue__JKI_lib_State_Machine.vi"("State(s) in (\"\")"=w348) -> ("States Out"=w349:string)  [unwired: 14 in]
      }
      frame "UI: Update Mermaid" {
        n140 = Unbundle By Name(w359) -> ("Mermaid.string"=w354:string, "Mermaid.Template"=w357:string, "Mermaid.output path"=w358:path)
        "mermaid string" <- w354
        n141 = feedback-in #2(w354) -> ()
        n142 = feedback #2("" ("string")) -> (w355:string)
        n143 = Not Equal?(x=w354, y=w355) -> (x != y?=w353:bool)
        n144 = case shown="True" w353 {
          tunnel: w358 -> [_ w370]
          tunnel: w357 -> [_ w368]
          tunnel: w354 -> [_ w365]
          frame False {
          }
          frame True {
            n145 = Search and Replace String(input string=w368, search string="%s", replace string=w365) -> (result string=w366:string)  [unwired: 5 in, 3 out]
            n146 = Text to UTF-8(11:w366) -> (3:w369:string)  [unwired: 2 in, 1 out]
            n147 = Write to Text File(file (use dialog)=w370, text=w369) -> ()  [unwired: 2 in, 3 out]
            n148 = Path To String(path=w370) -> (string=w364:string)
            n149 = invoke on="WebView2 Control" class="WebView2 Control (strict)" method="Navigate And Wait.vi"("Source"=w364, "Timeout (Inf)"=2000) -> ()  [unwired: 5 in, 7 out]
          }
        }
      }
      frame "UI: Update Toolbar" {
        n150 = Unbundle By Name(w376) -> ("Core.Current VI Reference"=w375:refnum<vi>, "LogFile"=w372:path)  [unwired: 1 out]
        n151 = Empty String/Path?(string/path=w372) -> (empty?=w371:bool)
        n152 = case shown="True" w371 {
          tunnel: "Running Log Viewer (CSM)" ("Front Panel Window:Title") -> [w384 w385]
          tunnel: [w383 w385] -> w373
          tunnel: w372 -> [w380 _]
          frame False {
            n153 = Path To String(path=w380) -> (string=w381:string)
            n154 = Concatenate Strings(w384, " - " ("string"), w381) -> (w383:string)
          }
          frame True {
          }
        }
        n155 = property class="VI"(reference=w375, "Front Panel.Title"=w373) -> ()  [unwired: 1 in, 2 out]
      }
      frame "UI: Resize Tab Content" {
        n156 = control-ref of="Tab"() -> (w394:refnum<vi>)
        n157 = control-ref of="Sub Panel"() -> (w395:refnum<vi>)
        n158 = control-ref of="mermaid string"() -> (w393:refnum<vi>)
        n159 = invoke class="TabCtl (strict)" method="FitControlToPane"(reference=w394) -> (reference out=w391:refnum<vi>)  [unwired: 2 in, 2 out]
        n160 = Build Array(w393, w395) -> (w392:refnum<vi>[])
        n161 = for {
          tunnel: w392 -> [w403] mode=indexing
          tunnel: w391 -> [w402]
          tunnel: [w401] -> w390
          n162 = call <userlib>:"Fit Control to Tab.vi"("Control"=w403, "TabRef"=w402) -> ("Rect"=w401:T15)  [unwired: 5 in, 2 out]
        }
        n163 = control-ref of="WebView2 Control"() -> (w396:refnum<vi>)
        n164 = Unbundle By Name(w390) -> ("Left"=w389:i32, "Right"=w388:i32, "Height"=w387:i32, "Width"=w386:i32)
        n165 = property class="WebView2 Control (strict)"(reference=w396, "Left"=w389, "Top"=w388, "Height"=w387, "Width"=w386) -> ()  [unwired: 1 in, 2 out]
      }
      frame "---------- Macro ----------" {
        # "Do not put any code in this frame.\n(It is a separator no-op. You can make a copy of this frame to create a new Macro frame)"
        n166 = call <vilib>:"Add State(s) to Queue__JKI_lib_State_Machine.vi"("State(s) in (\"\")"=w408) -> ("States Out"=w407:string)  [unwired: 14 in]
      }
      frame "Macro: Initialize" {
        # "Initialization Macro\n(This is called once, when the VI starts)"
        n167 = call <vilib>:"Add State(s) to Queue__JKI_lib_State_Machine.vi"("State(s) in Front (\"\")"="Data: Initialize\nData: Initialize References\nInitialize Core Data\nUI: Initialize\nUI: Front Panel State >> Open\nUI: Resize Tab Content\nAction: Start Registration Console\nUI: Refresh CSM List\nUI: Update Toolbar\nUI: Update Broadcast Registry\nMermaid: Update Broadcast Registry\nUI: Update Mermaid", "State(s) in (\"\")"=w414) -> ("States Out"=w413:string)  [unwired: 13 in]
      }
      frame "Macro: Exit" {
        # "Exit Macro\n(This is called once, when the VI exits)"
        n168 = Unbundle By Name(w419) -> ("Core.Close Panel on Exit?"=w431:bool)
        n169 = Unbundle By Name(w419) -> ("Mermaid.output path"=w424:path)
        n170 = Concatenate Strings(w415, ".*") -> (w416:string)
        n171 = call <userlib>:"_Broadcast Message.vi"("Module Pattern (support *)"=w416, "Broadcast"=_BroadcastDef."Macro: Exit") -> ()  [unwired: 9 in, 1 out]
        n172 = call <vilib>:"Check if File or Folder Exists.vi"("path"=w424) -> ("error out"=w423:errorcluster, "file or folder exists?"=w420:bool, "dup path"=w422:path)  [unwired: 8 in]
        n173 = case shown="True" w420 {
          tunnel: w423 -> [w435 w438]
          tunnel: w422 -> [_ w437]
          tunnel: [w435 w436] -> w421
          frame False {
          }
          frame True {
            n174 = Delete(path (use dialog)=w437, error in=w438) -> (error out=w436:errorcluster)  [unwired: 3 in, 2 out]
          }
        }
        n175 = call <vilib>:"Clear Errors.vi"("error in (no error)"=w421) -> ()  [unwired: 5 in, 2 out]
        n176 = Select(t="//UI: Front Panel State >> Close", s=w431, f="") -> (s? t:f=w428:string)
        n177 = call <vilib>:"Add State(s) to Queue__JKI_lib_State_Machine.vi"("State(s) in (\"\")"=w428, "State(s) at Back (\"\")"="Data: Cleanup\nExit") -> ("States Out"=w426:string)  [unwired: 13 in]
        n178 = call <vilib>:"Add State(s) to Queue__JKI_lib_State_Machine.vi"("State(s) in Front (\"\")"=w426, "State(s) in (\"\")"=w434) -> ("States Out"=w433:string)  [unwired: 13 in]
      }
      frame "----------- Mermaid ------------" {
      }
      frame "Mermaid: Update Broadcast Registry" {
        n179 = call "Generate Status-API Mapping mermaid.vi"() -> ("String"=w443:string)  [unwired: 9 in, 2 out]
        n180 = Bundle By Name(cluster=w448, "Mermaid.string"=w443) -> (w446:T12)
        n181 = call <vilib>:"Add State(s) to Queue__JKI_lib_State_Machine.vi"("State(s) in (\"\")"=w444) -> ("States Out"=w445:string)  [unwired: 14 in]
      }
      frame "Mermaid: Update All CSM Interface" {
        n182 = call <userlib>:"CSM - List Modules.vi"() -> ("error out"=w456:errorcluster, "Module Names"=w455:string[])  [unwired: 10 in]
        n183 = for {
          tunnel: [w474] -> w458 mode=indexing if=w468
          tunnel: w457 -> [w473]
          tunnel: w455 -> [w470] mode=indexing
          tunnel: w456 -> [w471]
          n184 = call "Query VIRef with Error Cache.vi"("Current Module(\"\" to generate a ID)"=w473, "Error In (no error)"=w471, "Target Module"=w470) -> ("error out"=w472:errorcluster, "CSM VI Ref"=w463:refnum<vi>)  [unwired: 7 in]
          n185 = call-poly <userlib>:"CSM-Helper API.vi"("error in (no error)"=w472, "VI"=w463) -> ("error out"=w466:errorcluster, "CSM-Helper.lvclass"=w467:refnum<class "CSM-Helper.lvclass">)  [unwired: 8 in]
          n186 = call "Generate CSM Class mermaid(CSMH).vi"("error in (no error)"=w466, "CSM-Helper in"=w467) -> ("error out"=w465:errorcluster, "resulting string"=w474:string, "CSM-Helper out"=w464:refnum<class "CSM-Helper.lvclass">)  [unwired: 7 in]
          n187 = call-poly <userlib>:"CSM-Helper API.vi"("error in (no error)"=w465, "CSM-Helper in"=w464) -> ("error out"=w469:errorcluster)  [unwired: 8 in, 1 out]
          n188 = Not(x=w469) -> (.not. x?=w468:bool)
        }
        n189 = Build Array (concatenate)("classDiagram\ndirection LR", w458) -> (w452:string[])
        n190 = call <userlib>:"1D Array to String_csm.vi"("delimiter (Tab)"="\r", "Array of Strings"=w452) -> ("delimited string"=w454:string)  [unwired: 9 in]
        n191 = Bundle By Name(cluster=w461, "Mermaid.string"=w454) -> (w459:T12)
      }
      frame "Mermaid: Update CSM Interface" {
        n192 = local read "CSM"() -> (w476:string)
        n193 = call "Query VIRef with Error Cache.vi"("Current Module(\"\" to generate a ID)"=w488, "Target Module"=w476) -> ("error out"=w482:errorcluster, "CSM VI Ref"=w475:refnum<vi>)  [unwired: 8 in]
        n194 = call-poly <userlib>:"CSM-Helper API.vi"("error in (no error)"=w482, "VI"=w475) -> ("error out"=w480:errorcluster, "CSM-Helper.lvclass"=w481:refnum<class "CSM-Helper.lvclass">)  [unwired: 8 in]
        n195 = call "Generate CSM Class mermaid(CSMH).vi"("error in (no error)"=w480, "CSM-Helper in"=w481) -> ("error out"=w479:errorcluster, "resulting string"=w489:string, "CSM-Helper out"=w478:refnum<class "CSM-Helper.lvclass">)  [unwired: 7 in]
        n196 = call-poly <userlib>:"CSM-Helper API.vi"("error in (no error)"=w479, "CSM-Helper in"=w478) -> ("error out"=w477:errorcluster)  [unwired: 8 in, 1 out]
        n197 = Build Array("classDiagram\ndirection LR", w489) -> (w485:string[])
        n198 = call <vilib>:"Clear Errors.vi"("error in (no error)"=w477) -> ()  [unwired: 5 in, 2 out]
        n199 = call <userlib>:"1D Array to String_csm.vi"("delimiter (Tab)"="\r", "Array of Strings"=w485) -> ("delimited string"=w487:string)  [unwired: 9 in]
        n200 = Bundle By Name(cluster=w492, "Mermaid.string"=w487) -> (w490:T12)
      }
      frame "Action: Start Registration Console" {
        n201 = vi-ref <userlib>:"Registration Console.vi"() -> (w500:refnum<vi>)
        n202 = property class="VI Interface Type 0"(reference=w500) -> (reference out=w506:refnum<vi>, error out=w505:errorcluster, "Path"=w504:path)  [unwired: 1 in]
        n203 = Open VI Reference(type specifier VI Refnum (for type only)=w506, vi path=w504, options=128, error in (no error)=w505) -> (vi reference=w496:refnum<vi>, error out=w503:errorcluster)  [unwired: 2 in]
        n204 = call <userlib>:"Concatenate Submodule Name.vi"("Module Name"="RegConsole", "Group Name"=w494) -> ("Submodule Name"=w499:string)  [unwired: 9 in]
        n205 = call-by-ref "Start Asynchronous Call"(reference=w496, error in=w503, "name"=w499) -> (reference out=w501:refnum<vi>, error out=w507:errorcluster)  [unwired: 11 in]
        n206 = control-ref of="Sub Panel"() -> (w497:refnum<vi>)
        n207 = Close Reference(reference=w501, error in (no error)=w507) -> (error out=w495:errorcluster)
        n208 = invoke on="Invoke Node" class="SubPnl" method="Insert VI"(reference=w497, error in=w495, "VI Ref"=w496) -> ()  [unwired: 1 in, 4 out]
      }
    }
  }
  n209 = control-ref of="Current VI Reference"() -> (w1:refnum<vi>)
  n210 = call <userlib>:"CSM - Destroy Global Log Event.vi"("Error In"=w5, "CSM Global Log Event"=w11) -> ("error out"=w2:errorcluster)  [unwired: 9 in]
  n211 = call <userlib>:"Close FP if in LabVIEW Dir.vi"("VI Refnum"=w1, "Error in"=w2) -> ("Error out"=w3:errorcluster)  [unwired: 9 in]
  n212 = call <vilib>:"Clear Errors.vi"("error in (no error)"=w3) -> ()  [unwired: 5 in, 2 out]
